vi "Setup Telem APIs.vi"(8 "error in (no error)":errorcluster, 11 "Volatus Core in":refnum<class "Volatus Core.lvclass">) -> (0 "error out":errorcluster, 3 "Volatus Core out":refnum<class "Volatus Core.lvclass">)   [LabVIEW 2020, in "Volatus.lvlib" / "Volatus Core.lvclass"]
uses:
  Volatus Core.lvclass
  C:/dev/lv20CE/relink/lv-volatus/Volatus/Module/Module.lvclass
  Volatus Core.lvclass/Volatus Core.ctl
  Module/Module.lvclass/Module.ctl
  VolatusAPI/VolatusAPI.lvclass/VolatusAPI.ctl
  Module/Module.lvclass
  lv-vecto/Vecto/Vecto/Vecto.lvclass
  VolatusAPI/VolatusAPI.lvclass
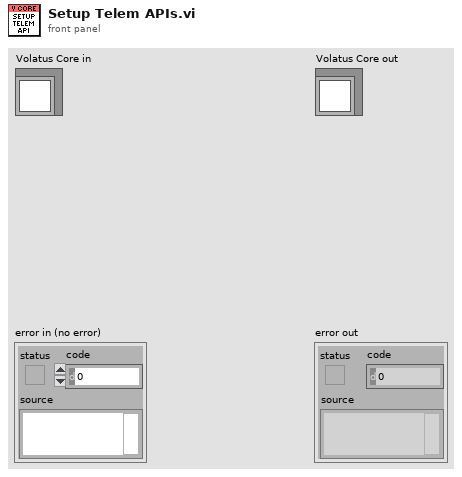
[diagram p1: front panel]
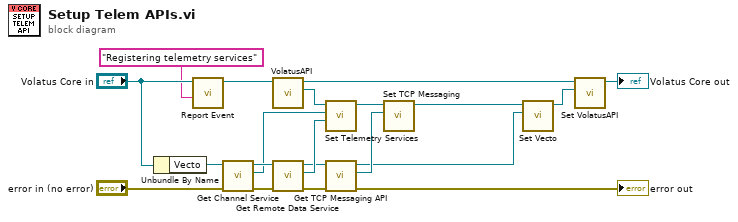
[diagram p0: block diagram]
diagram:
  n1 = Unbundle By Name("Volatus Core in") -> ("Vecto"=w18:refnum<class "Vecto.lvclass">)
  n2 = call "Report Event.vi"("Message"="Registering telemetry services", "Module in"="Volatus Core in") -> ("Module out"=w9:refnum<class "Volatus Core.lvclass">)  [unwired: 8 in, 1 out]
  n3 = call "Get Channel Service.vi"("error in (no error)"="error in (no error)", "Vecto in"=w18) -> ("error out"=w13:errorcluster, "ChannelService"=w15:refnum<class "ChannelService.lvclass">, "Vecto out"=w20:refnum<class "Vecto.lvclass">)  [unwired: 7 in]
  n4 = call "VolatusAPI.vi"("Module in"=w9) -> ("VolatusAPI"=w16:refnum<class "VolatusAPI.lvclass">, "Module out"=w17:refnum<class "Volatus Core.lvclass">)  [unwired: 9 in]
  n5 = call "Get Remote Data Service.vi"("error in (no error)"=w13, "Vecto in"=w20) -> ("error out"=w6:errorcluster, "RemoteDataService"=w14:refnum<class "RemoteDataService.lvclass">, "Vecto out"=w5:refnum<class "Vecto.lvclass">)  [unwired: 7 in]
  n6 = call "Set Telemetry Services.vi"("RemoteDataService"=w14, "ChannelService"=w15, "VolatusAPI in"=w16) -> ("VolatusAPI out"=w10:refnum<class "VolatusAPI.lvclass">)  [unwired: 8 in]
  n7 = call "Get TCP Messaging API.vi"("error in (no error)"=w6, "Vecto in"=w5) -> ("error out"=→"error out":errorcluster, "TCP Messaging API"=w4:refnum<class "TCPMessageAPI.lvclass">, "Vecto out"=w1:refnum<class "Vecto.lvclass">)  [unwired: 7 in]
  n8 = call "Set TCP Messaging.vi"("Messaging"=w4, "VolatusAPI in"=w10) -> ("VolatusAPI out"=w7:refnum<class "VolatusAPI.lvclass">)  [unwired: 8 in, 1 out]
  n9 = call "Set Vecto.vi"("Vecto"=w1, "VolatusAPI in"=w7) -> ("VolatusAPI out"=w2:refnum<class "VolatusAPI.lvclass">)  [unwired: 9 in]
  n10 = call "Set VolatusAPI.vi"("VolatusAPI"=w2, "Module in"=w17) -> ("Module out"=→"Volatus Core out":refnum<class "Volatus Core.lvclass">)  [unwired: 9 in]
